vi "SLSC Enable Buttons.vi"(8 "error in (no error)":errorcluster, 11 "data":T1) -> (0 "error out":errorcluster)   [LabVIEW 2020, in "SLSC EDS System Explorer.lvlib"]
uses:
  System Explorer/SLSC EDS System Explorer.lvlib
  SLSC EDS API/JSON parsing/EDSjsonStructure.ctl
  SLSC EDS API/JSON parsing/enum.ctl
  SLSC EDS API/JSON parsing/property.ctl
  SLSC EDS API/JSON parsing/command.ctl
  SLSC EDS API/JSON parsing/scale.ctl
  SLSC EDS API/JSON parsing/physicalChannel.ctl
  SLSC EDS API/JSON parsing/register.ctl
  <vilib>/NI VeriStand/Custom Device API/Custom Device API.lvlib
panel:
  # "not working\nregisterMap->registers->initialValue"
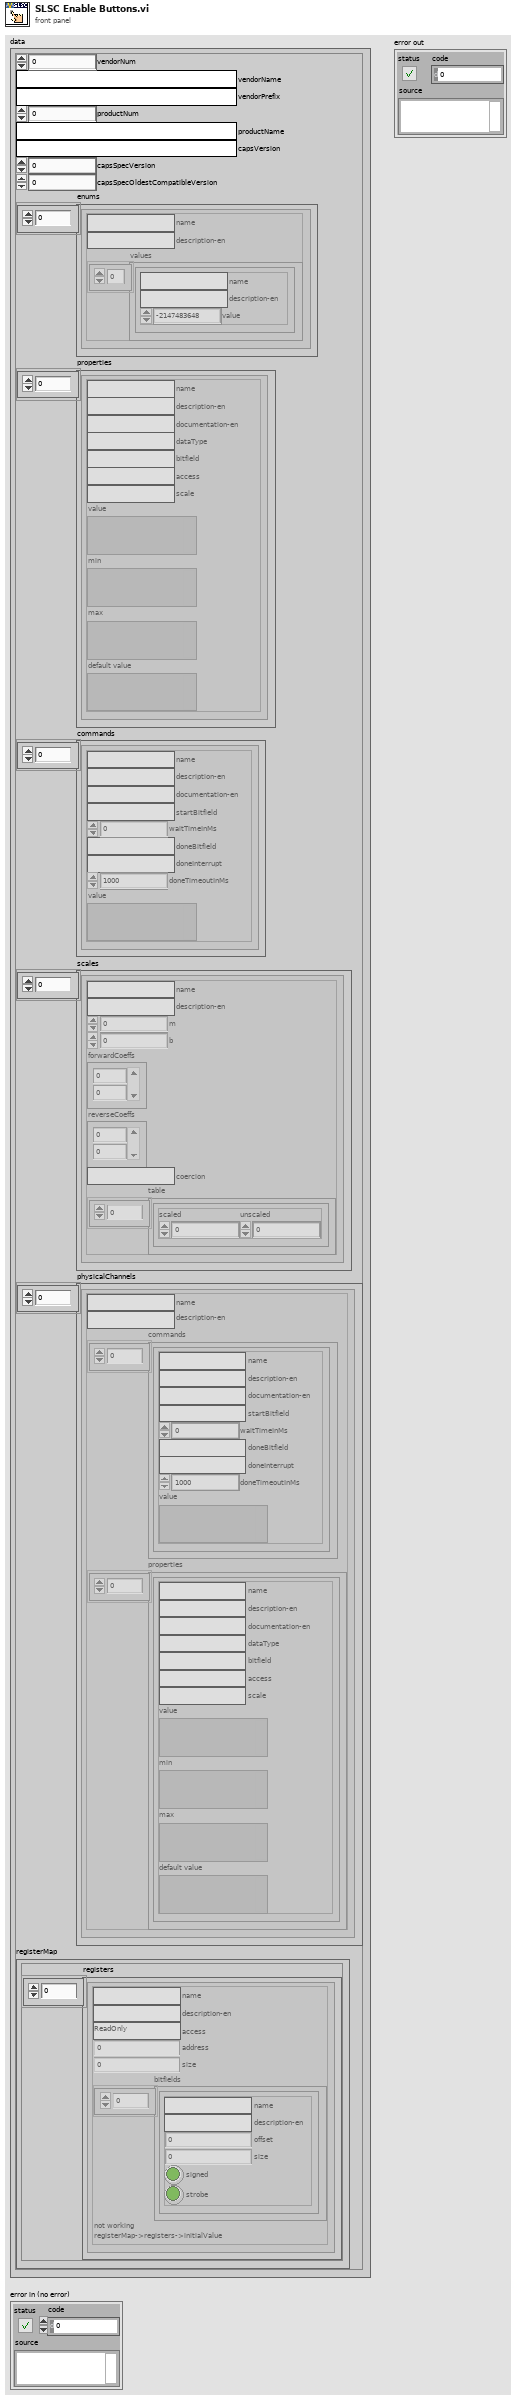
[diagram p1: front panel]
types:
  T1 = typedef "EDSjsonStructure.ctl" = cluster{"vendorNum":u32, "vendorName":string, "vendorPrefix":string, "productNum":u32, "productName":string, "capsVersion":string, "capsSpecVersion":u32, "capsSpecOldestCompatibleVersion":u32, "enums":T2[], "properties":T3[], "commands":T4[], "scales":T5[], "physicalChannels":T6[], "registerMap":cluster{"registers":T7[]}}
  T2 = typedef "enum.ctl" = cluster{"name":string, "description-en":string, "values":cluster{"name":string, "description-en":string, "value":i32}[]}
  T3 = typedef "property.ctl" = cluster{"name":string, "description-en":string, "documentation-en":string, "dataType":string, "bitfield":string, "access":string, "scale":string, "value":variant, "min":variant, "max":variant, "default value":variant}
  T4 = typedef "command.ctl" = cluster{"name":string, "description-en":string, "documentation-en":string, "startBitfield":string, "waitTimeInMs":i32, "doneBitfield":string, "doneInterrupt":string, "doneTimeoutInMs":i32, "value":variant}
  T5 = typedef "scale.ctl" = cluster{"name":string, "description-en":string, "m":dbl, "b":dbl, "forwardCoeffs":dbl[], "reverseCoeffs":dbl[], "coercion":string, "table":cluster{"scaled":dbl, "unscaled":dbl}[]}
  T6 = typedef "physicalChannel.ctl" = cluster{"name":string, "description-en":string, "commands":T4[], "properties":T3[]}
  T7 = typedef "register.ctl" = cluster{"name":string, "description-en":string, "access":string, "address":u32, "size":u32, "bitfields":cluster{"name":string, "description-en":string, "offset":u32, "size":u32, "signed":bool, "strobe":bool}[]}
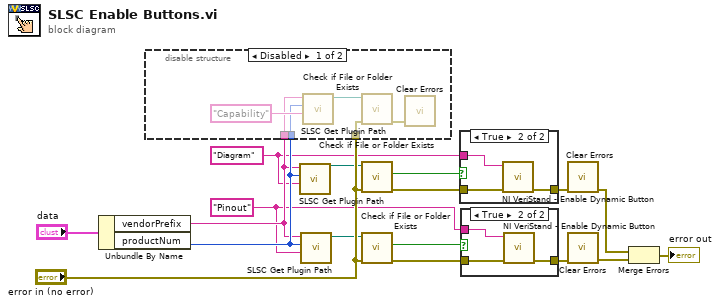
[diagram p0: block diagram]
diagram:
  w7 = "Diagram" ("Type")
  w9 = "Pinout" ("Type")
  n1 = Unbundle By Name("data") -> ("vendorPrefix"=w15:string, "productNum"=w16:u32)
  n2 = disable-structure shown="Disabled" {
    disable-tunnel: "error in (no error)" -> [w22 _]
    disable-tunnel: w16 -> [w19 _]
    disable-tunnel: w15 -> [w18 _]
    frame Disabled {
      n3 = call "SLSC Get Plugin Path.vi"("Type"="Capability", "number"=w19, "Vendor Prefix"=w18) -> ("appended path"=w21:path)  [unwired: 8 in]
      n4 = call <vilib>:"Check if File or Folder Exists.vi"("error in (no error)"=w22, "path"=w21) -> ("error out"=w23:errorcluster)  [unwired: 7 in, 2 out]
      n5 = call <vilib>:"Clear Errors.vi"("error in (no error)"=w23) -> ()  [unwired: 1 in, 6 out]
    }
    frame Enabled {
    }
  }
  n6 = call "SLSC Get Plugin Path.vi"("Type"=w7, "number"=w16, "Vendor Prefix"=w15) -> ("appended path"=w5:path)  [unwired: 8 in]
  n7 = call "SLSC Get Plugin Path.vi"("Type"=w9, "number"=w16, "Vendor Prefix"=w15) -> ("appended path"=w6:path)  [unwired: 8 in]
  n8 = call <vilib>:"Check if File or Folder Exists.vi"("error in (no error)"="error in (no error)", "path"=w5) -> ("error out"=w11:errorcluster, "file or folder exists?"=w8:bool)  [unwired: 7 in, 1 out]
  n9 = call <vilib>:"Check if File or Folder Exists.vi"("error in (no error)"="error in (no error)", "path"=w6) -> ("error out"=w12:errorcluster, "file or folder exists?"=w10:bool)  [unwired: 7 in, 1 out]
  n10 = case shown="True" w8 {
    tunnel: w7 -> [_ w27]
    tunnel: w11 -> [w24 w26]
    tunnel: [w24 w25] -> w13
    frame False {
    }
    frame True {
      n11 = call <vilib>:"NI VeriStand - Enable Dynamic Button.vi"("error in (no error)"=w26, "Button ID"=w27) -> ("error out"=w25:errorcluster)  [unwired: 9 in]
    }
  }
  n12 = case shown="True" w10 {
    tunnel: w9 -> [_ w31]
    tunnel: w12 -> [w28 w30]
    tunnel: [w28 w29] -> w14
    frame False {
    }
    frame True {
      n13 = call <vilib>:"NI VeriStand - Enable Dynamic Button.vi"("error in (no error)"=w30, "Button ID"=w31) -> ("error out"=w29:errorcluster)  [unwired: 9 in]
    }
  }
  n14 = call <vilib>:"Clear Errors.vi"("error in (no error)"=w13) -> ("error out"=w2:errorcluster)  [unwired: 1 in, 5 out]
  n15 = call <vilib>:"Clear Errors.vi"("error in (no error)"=w14) -> ("error out"=w3:errorcluster)  [unwired: 1 in, 5 out]
  n16 = Merge Errors(w2, w3) -> (→"error out":errorcluster)
